vi "Stop Condition - Saturation 2 (SubVI) (1).vi"(6 "Enum":enum16{"Saturation", "Sat Step", "Sat Ramp"}(ring), 8 "error in (no error)":errorcluster, 9 "Test RunTime":dbl, 10 "Time":dbl, 11 "Cluster in":T1 {"M Event" items=["Stop", "Running", "PID", "Up Limit", "Down Limit", "Load Limit"]; "Test Type" items=["Please Select", "Triaxial Shear", "Triaxial UU", "Shearbox", "Permeability", "Consolidation (Stepped Loading)/Swelling", "Saturation (Incremental)", "User Defined", "UCT", "Isotropic Consolidation", "Swelling Pressure", "B-Check", "Saturation (Step Increment)", "Saturation (Ramp)"]; "Data"."Test Type" items=["Please Select", "Triaxial Shear", "Triaxial UU", "Shearbox", "Permeability", "Consolidation (Stepped Loading)/Swelling", "Saturation (Incremental)", "User Defined", "UCT", "Isotropic Consolidation", "Swelling Pressure", "B-Check", "Saturation (Step Increment)", "Saturation (Ramp)"]}) -> (0 "error out":errorcluster, 3 "Cluster out":T1 {"M Event" items=["Stop", "Running", "PID", "Up Limit", "Down Limit", "Load Limit"]; "Test Type" items=["Please Select", "Triaxial Shear", "Triaxial UU", "Shearbox", "Permeability", "Consolidation (Stepped Loading)/Swelling", "Saturation (Incremental)", "User Defined", "UCT", "Isotropic Consolidation", "Swelling Pressure", "B-Check", "Saturation (Step Increment)", "Saturation (Ramp)"]; "Data"."Test Type" items=["Please Select", "Triaxial Shear", "Triaxial UU", "Shearbox", "Permeability", "Consolidation (Stepped Loading)/Swelling", "Saturation (Incremental)", "User Defined", "UCT", "Isotropic Consolidation", "Swelling Pressure", "B-Check", "Saturation (Step Increment)", "Saturation (Ramp)"]}, 4 "Delay":string, 7 "Log?":bool)   [LabVIEW 2019]
uses:
  Controls/RunTest - Data Structure.ctl
  Controls/Test Panel - Data Structure.ctl
  Controls/Station - Test Type.ctl
  <vilib>/Utility/miscctls.llb/LVRowAndColumnTypeDef.ctl
  Controls/RunTest - Calculate Data.ctl
  <vilib>/httpClient/ClientHandle.ctl
  Controls/RunTest - Start Condition.ctl
  Controls/RunTest - Stop Condition.ctl
  Controls/UDP - Event.ctl
  Controls/eFGV States.ctl
  <vilib>/httpClient/LabVIEWHTTPClient.lvlib
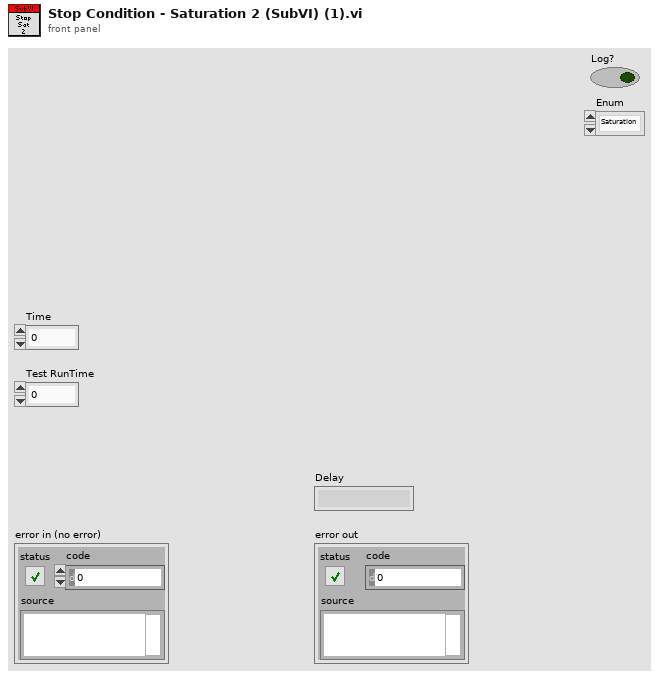
[diagram p1: front panel]
types:
  T1 = typedef "RunTest - Data Structure.ctl" = cluster{"Test Plan":string[], "PlanRow":i32, "Device Name":string[], "Timeout":i32, "Start?":bool, "Pause?":bool, "IP Address":string[], "LogRow":i32, "Logtype":u16, "Log Elapse":sgl, "Data":T2, "Stop log?":bool, "tdms":refnum<k34>, "Sensor Data":sgl[], "Start time":timestamp, "Prev Log Elapse":u32, "Plot":u16, "X-Axis":u16[], "Y-Axis":u16[], "XY":cluster{"X":dbl, "Y":dbl}[][], "End Stage?":bool, "1run":bool, "Condition":u16[], "Start Con":bool, "Log Con":bool, "Stop Con":bool, "Start Elapse":dbl, "Start Load":dbl, "Motor":i32, "StartRow":i32, "number log":i32, "Dir":bool, "Start time test":timestamp, "Auto":bool, "Check return?":bool, "Inv":cluster{"M":i32[], "Bool":bool[]}, "tdms temp":refnum<k34>, "Zero?":bool, "Plot Timer":dbl, "1st Run":bool, "TDMS Path":path, "MaxLoad":dbl, "Log Timer":sgl[], "Test Type":T3, "Log Sensor":string[], "Save?":bool, "1st Log":bool, "Y-Axis 2":u16[], "On Y-Axis 2":bool, "Decimal":u8[], "Init":cluster{"PWP TS":sgl, "Load TS":sgl, "Volume TS":sgl, "Disp TS":sgl, "CP":sgl, "Vol In":sgl, "Vol Out":sgl, "Load UCT":sgl, "Disp UCT":sgl, "PWP Sat":sgl, "CP Sat":sgl, "Volume IsoCons":sgl, "PWP IsoCons":sgl, "PWP TUU":sgl, "Load TUU":sgl, "Volume TUU":sgl, "Disp TUU":sgl, "Load Cons":sgl, "Disp Cons":sgl, "Volume Sat":sgl, "Vertical Load SB":sgl, "Vertical Disp SB":sgl, "H Disp SB":sgl, "H Load SB":sgl, "PWP BC":sgl, "CP BC":sgl, "PWP Sat Step":sgl, "CP Sat Step":sgl, "Volume Sat Step":sgl, "PWP Sat Ramp":sgl, "CP Sat Ramp":sgl, "Volume Sat Ramp":sgl}, "Calc":T5, "Device Index":i32[], "Channel Index":i32[], "http ref":T6, "fileid":string, "Step Cons":cluster{"V Stress":sgl, "H Settlement":sgl}, "RunTest":bool, "Graph Last":i32, "Init?":bool, "Datalog":bool[], "Start":T7, "Stop":T8, "Running?":bool, "StartTime":dbl, "Log Prev Time":dbl, "KeyName":string[], "Test RunTime":dbl, "Log Prev Axial":dbl, "M Event":T9[], "Last Log":bool, "popup":bool, "PreStart UU":bool, "PreStart Sat":bool, "PreStart BC":bool, "PreStart Sat Step":bool, "PreStart Sat Ramp":bool, "Prev Sat IP":string}
  T2 = typedef "Test Panel - Data Structure.ctl" = cluster{"Station":string, "Sample ID":string, "Job No":string, "Job Description":string, "Filename":string, "Test Type":T3, "Speciment No":string, "Depth":string, "Height":string, "Diameter/Length":string, "Weight":string, "Test Parameter":string, "Station[]":string[], "Edit Pos":T4, "Edit Pos Prev":T4, "Area":string, "Path":string, "sample_id":string}
  T3 = typedef "Station - Test Type.ctl" = u16
  T4 = typedef "LVRowAndColumnTypeDef.ctl" = cluster{"Row":i32, "Column":i32}
  T5 = typedef "RunTest - Calculate Data.ctl" = cluster{"TS":cluster{"Change PWP":sgl, "Change Vol":sgl, "Axial Load":sgl, "CiL":sgl, "Deviator":sgl, "Axial Strain":sgl, "MaxDeviator":sgl, "SS":sgl, "CAS":sgl}, "TUU":cluster{"Change PWP":sgl, "Axial Load":sgl, "CiL":sgl, "Deviator":sgl, "Axial Strain":sgl, "MaxDeviator":sgl}, "Sat":cluster{"B Value":sgl, "PWP Diss":sgl, "CPP":sgl, "CV":sgl}, "Per":cluster{"Change Vol In":sgl, "Change Vol Out":sgl, "Mean Vol":sgl, "Gradient Pressure":sgl, "Outlet Flow":sgl, "Inlet Flow":sgl, "I X1":sgl, "I X2":sgl, "I Y1":sgl, "I Y2":sgl, "O X1":sgl, "O X2":sgl, "O Y1":sgl, "O Y2":sgl}, "Step Cons":cluster{"V Stress":sgl, "H Settlement":sgl, "Total H Settle":sgl, "Prev Total H":sgl}, "UCT":cluster{"ALC":sgl, "H Change":sgl, "Deviator":sgl, "Axial Strain":sgl, "V Stress":sgl, "MaxDeviator":sgl}, "ISO Cons":cluster{"CPP":sgl, "PWP Diss":sgl, "CV":sgl, "VS":sgl}, "SB":cluster{"Speci LenC":sgl, "Shear Strain":sgl, "H LC":sgl, "Normal Stress":sgl, "Shear Stress":sgl, "MaxShear":sgl}, "BC":cluster{"B Value":sgl, "PWP Diss":sgl, "CPP":sgl, "CV":sgl}, "Sat Step":cluster{"B Value":sgl, "PWP Diss":sgl, "CPP":sgl, "CV":sgl}, "Sat Ramp":cluster{"B Value":sgl, "PWP Diss":sgl, "CPP":sgl, "CV":sgl}, "Prev Log":string[]}
  T6 = typedef "LabVIEWHTTPClient.lvlib/ClientHandle.ctl" = refnum<k1>
  T7 = typedef "RunTest - Start Condition.ctl" = cluster{"Cons":cluster{"VS":dbl, "Delay":bool, "No Delay":dbl}, "Sat":cluster{"CP":dbl, "BP":dbl, "StartBP":bool, "Target CP":bool, "Target BP":bool}, "Iso":cluster{"Select":dbl, "BP":dbl, "IC2":dbl, "IC3":dbl, "IC4":dbl, ". IC6":bool, "IC6":dbl, "IC6-2":dbl, "Time Cond":dbl, "Last PWP":dbl, "Target CP":bool, "Target BP":bool, "NewCP":dbl, "NewBP":dbl, "Noti CP":bool, "Noti BP":bool, "Noti PWP":bool, "PrevSatBP":dbl}, "TS":cluster{"SS":dbl, "Engage":bool, "ES":dbl, "LC":dbl, "PreStart":bool, "Trig SS":bool, "Drain":dbl, "Select":u16, "Max SS .":bool, "MaxSS":dbl}, "TUU":cluster{"SS":dbl, "Engage":bool, "ES":dbl, "LC":dbl, "PreStart":bool, "Trig SS":bool, "CP":dbl, "Delay Value":dbl, "Delay":bool, "CP PID":bool}, "UCT":cluster{"SS":dbl, "Engage":bool, "ES":dbl, "LC":dbl, "PreStart":bool, "Trig SS":bool}, "Enable?":bool, "SB":cluster{"SS":dbl, "Engage":bool, "ES":dbl, "LC":dbl, "PreStart":bool, "Trig SS":bool, "VS":dbl, "Delay Value":dbl, "Delay":bool, "VS PID":bool}, "Perm":cluster{"DP":dbl}, "BC":cluster{"CP":dbl, "Target CP":bool, "Target BP":bool, "CP Inc":dbl, "CP .Init":bool, "CP Init":dbl, "1st BC":bool}, "Sat (Step)":cluster{"Select":dbl, "CP":dbl, "BP":dbl, "EP":dbl, "StartCP":bool, "Target CP":bool, "Target BP":bool}, "Sat (Ramp)":cluster{"Select":dbl, "CP":dbl, "BP":dbl, "EP":dbl, "StartCP":bool, "Target CP":bool, "Target BP":bool, "Time Rate":u32}}
  T8 = typedef "RunTest - Stop Condition.ctl" = cluster{"Cons":cluster{"Select":i32, "Disp":dbl, "Time":dbl, "Time2":dbl, "Disp 2":dbl, "Time Cond":dbl, "Last Disp":dbl, "Swell":bool, "T50,90,100":cluster{"t50_x_min":dbl, "t50_y_value":dbl, "t90_x_min":dbl, "t90_y_value":dbl, "t100_x_min":dbl, "t100_y_value":dbl, "target_column":string, "test_type":string, "error":string}}, "Sat":cluster{"Select":i32, "PP":dbl, "Time":dbl, "VC":dbl, "Time2":dbl, "Time Cond":dbl, "Last PP":dbl, ".B":bool, "B":dbl, "Last Vc":dbl, "Time Cond 2":dbl, "Time3":dbl, "Time Cond 3":dbl, "B Achieve":bool, "PP Achieve":bool, "VC Achieve":bool, "Max Achieve":bool, "CP Check":dbl, "Skip Next":bool, "B Achieve Stage":u32, ".CP Check":bool}, "Iso":cluster{"PP":dbl, "Time":dbl, "VC":dbl, "Time2":dbl, "Time Cond":dbl, "Last Vc":dbl, ".PP":bool, "Time Cond 2":dbl, "Select":i32, "BS":cluster{"t50_x_min":dbl, "t50_y_value":dbl, "t90_x_min":dbl, "t90_y_value":dbl, "t100_x_min":dbl, "t100_y_value":dbl, "target_column":string, "test_type":string, "error":string}, "Final VC":dbl, "ASTM":cluster{"t50_x_min":dbl, "t50_y_value":dbl, "t90_x_min":dbl, "t90_y_value":dbl, "t100_x_min":dbl, "t100_y_value":dbl, "target_column":string, "test_type":string, "error":string}, "ASTM Log":cluster{"t50_x_min":dbl, "t50_y_value":dbl, "t90_x_min":dbl, "t90_y_value":dbl, "t100_x_min":dbl, "t100_y_value":dbl, "target_column":string, "test_type":string, "error":string}, "PP Achieve":bool, "VC Achieve":bool}, "TS":cluster{"Axial":dbl, ".MaxDev":bool, "MaxDev Value":dbl, "Return":bool, "Reset":bool, "Prev Time":dbl, "PostStop Run":bool, "CP Stop":bool, "BP Stop":bool, "PostStop Trig":bool, "Reset Value":dbl, "BPTrig":bool, "CPTrig":bool, "VLCTrig":bool, "CAxial":dbl, "Select":i32}, "TUU":cluster{"Axial":dbl, ".MaxDev":bool, "MaxDev Value":dbl, "Return":bool, "Reset":bool, "Prev Time":dbl, "PostStop Run":bool, "CP Stop":bool, "BP Stop":bool, "PostStop Trig":bool, "Reset Value":dbl, "BPTrig":bool, "CPTrig":bool, "VLCTrig":bool}, "UCT":cluster{"Axial":dbl, ".MaxDev":bool, "MaxDev Value":dbl, "Return":bool, "Reset":bool, "Prev Time":dbl, "PostStop Run":bool, "CP Stop":bool, "BP Stop":bool, "PostStop Trig":bool}, "Enable?":bool, "SB":cluster{"Shear":dbl, ".MaxShear":bool, "MaxShear Value":dbl, "Return":bool, "Reset":bool, "Prev Time":dbl, "PostStop Run":bool, "CP Stop":bool, "BP Stop":bool, "PostStop Trig":bool, "Reset Value":dbl, "BPTrig":bool, "CPTrig":bool, "VLCTrig":bool}, "Perm":cluster{"Max Time":bool, "Reset":bool, "PostStop Run":bool, "Ratio":bool, "Reset Value":dbl, "Time":dbl, "RatioTime":dbl, "RatioMore":dbl, "RatioLess":dbl, "Time Cond":dbl, "Time Cond 2":dbl, "Prev IF":dbl, "Prev OF":dbl, "PostStop Trig":bool, "BP Trig":bool, "DP Stop":bool, "BP Stop":bool, "CP Stop":bool, "CP Trig":bool}, "SP":cluster{".Max Time":bool, ".Time":bool, "Time":dbl, "MaxTime":dbl, "Time Cond":dbl, "Max Time Cond":dbl, "Stress":dbl}, "BC":cluster{"Select":i32, "PP":dbl, "Time":dbl, "Time Cond":dbl, "Last PP":dbl, ".B":bool, "B":dbl, "Time 2":dbl, "Time Cond 2":dbl, "B Achieve":bool, "PP Achieve":bool, "Max Achieve":bool, "CP Check":dbl, "Skip Next":bool, "B Achieve Stage":u32, ".CP Check":bool}, "Sat (Step)":cluster{"Select":i32, "PP":dbl, "Time":dbl, "VC":dbl, "Time2":dbl, "Time Cond":dbl, "Last PP":dbl, ".B":bool, "B":dbl, "Last Vc":dbl, "Time Cond 2":dbl, "Time3":dbl, "Time Cond 3":dbl, "B Achieve":bool, "PP Achieve":bool, "VC Achieve":bool, "Max Achieve":bool, "CP Check":dbl, "Skip Next":bool, "B Achieve Stage":u32}, "Sat (Ramp)":cluster{"Select":i32, "PP":dbl, "Time":dbl, "VC":dbl, "Time2":dbl, "Time Cond":dbl, "Last PP":dbl, ".B":bool, "B":dbl, "Last Vc":dbl, "Time Cond 2":dbl, "Time3":dbl, "Time Cond 3":dbl, "B Achieve":bool, "PP Achieve":bool, "VC Achieve":bool, "Max Achieve":bool, "CP Check":dbl, "Skip Next":bool, "B Achieve Stage":u32}}
  T9 = typedef "UDP - Event.ctl" = u16
  T10 = typedef "eFGV States.ctl" = enum16{"Init", "Read", "Write", "Exit"}
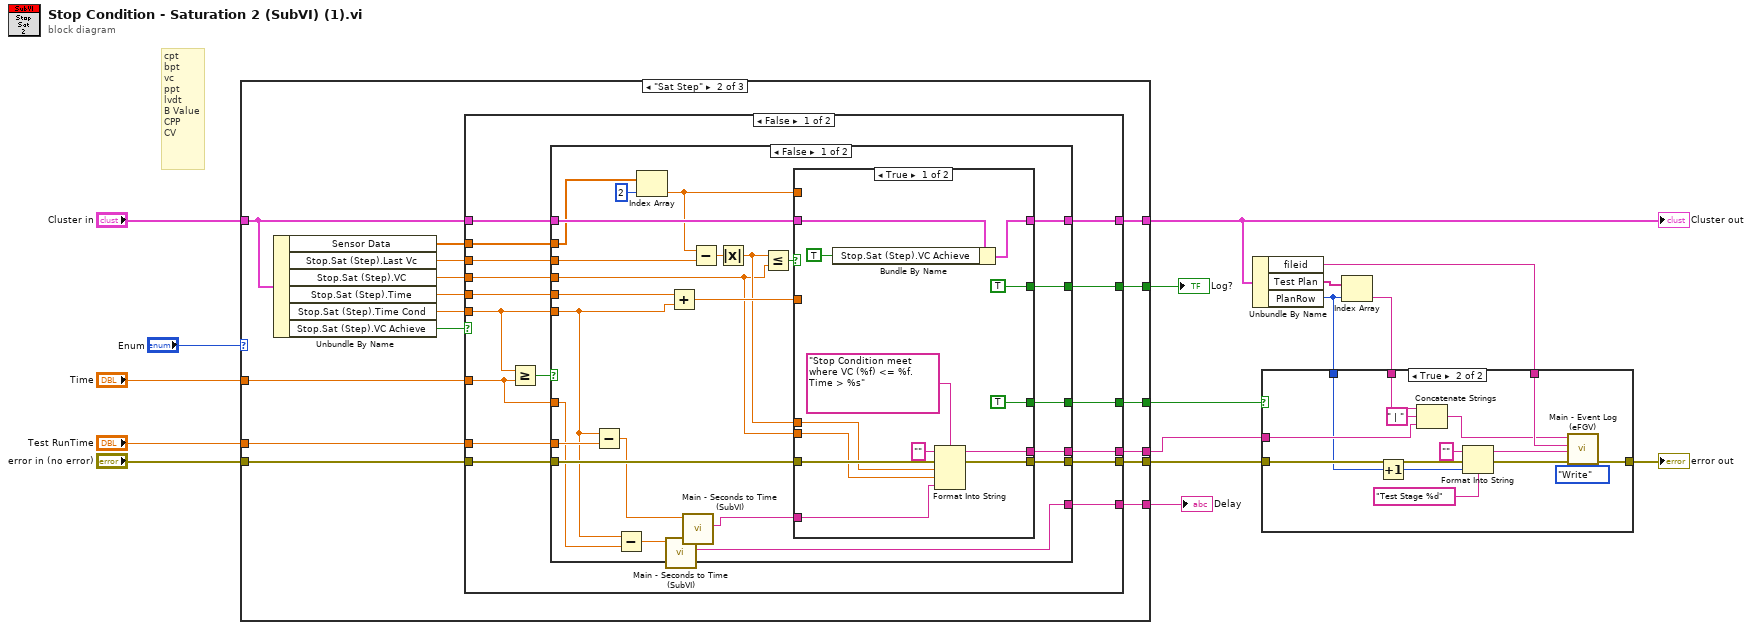
[diagram p0: block diagram]
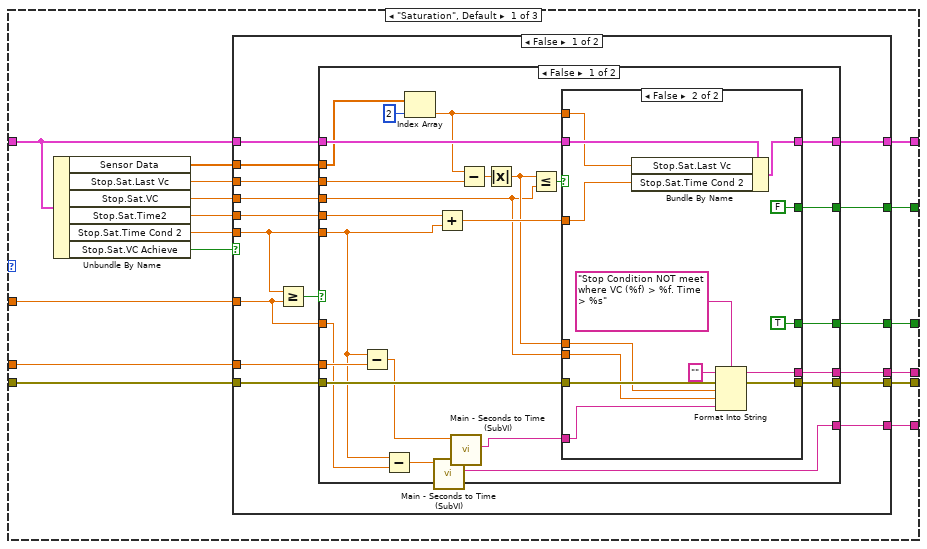
[diagram p2: hidden frame]
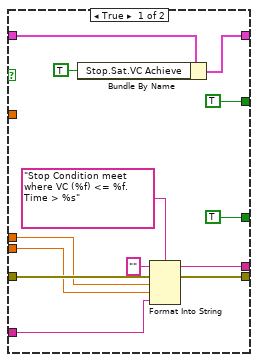
[diagram p3: hidden frame]
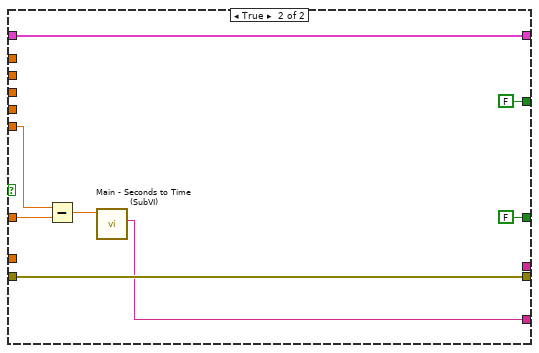
[diagram p4: hidden frame]
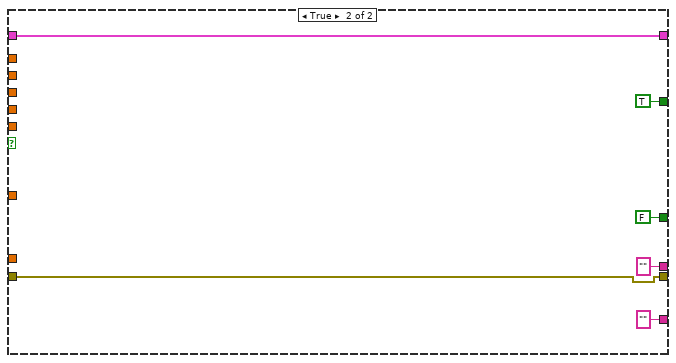
[diagram p5: hidden frame]
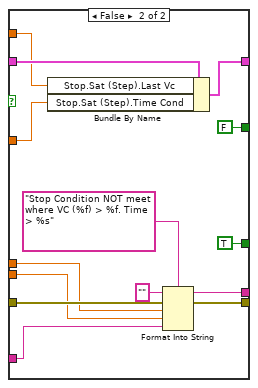
[diagram p6: hidden frame]
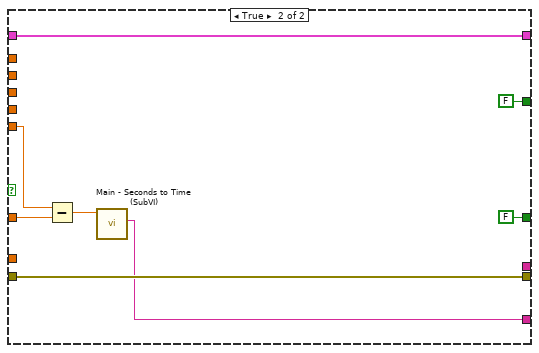
[diagram p7: hidden frame]
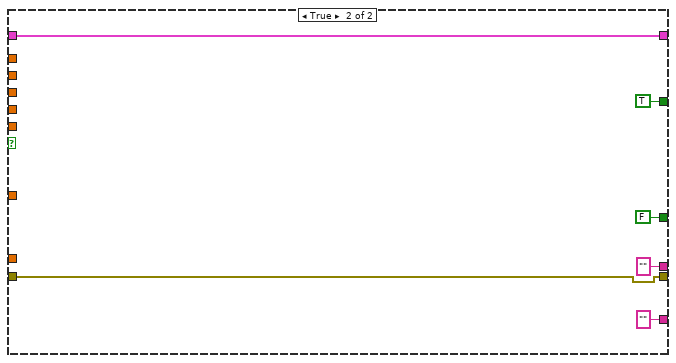
[diagram p8: hidden frame]
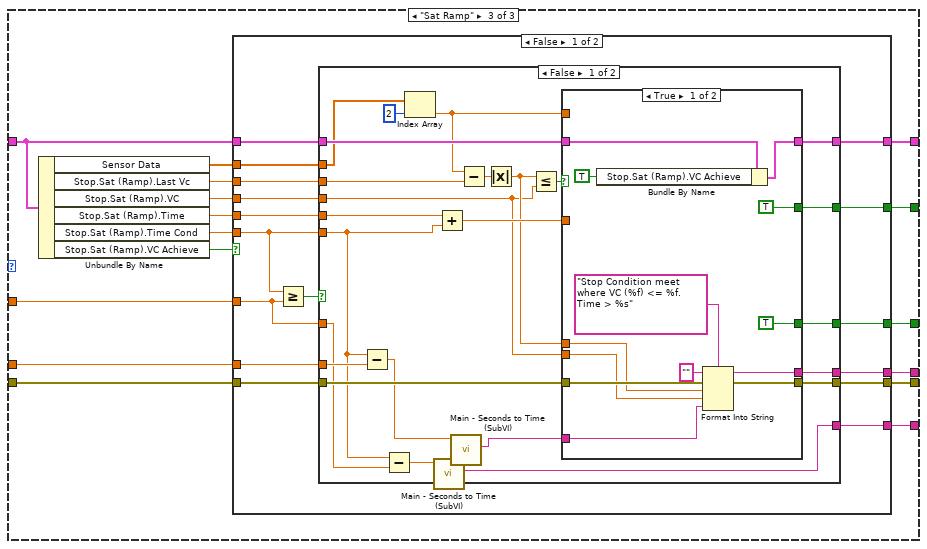
[diagram p9: hidden frame]
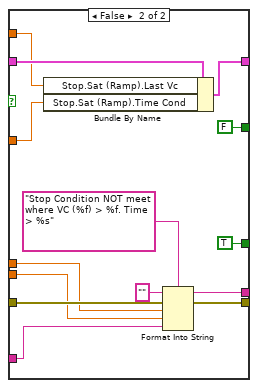
[diagram p10: hidden frame]
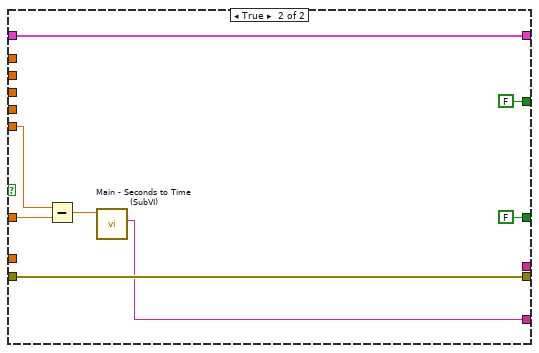
[diagram p11: hidden frame]
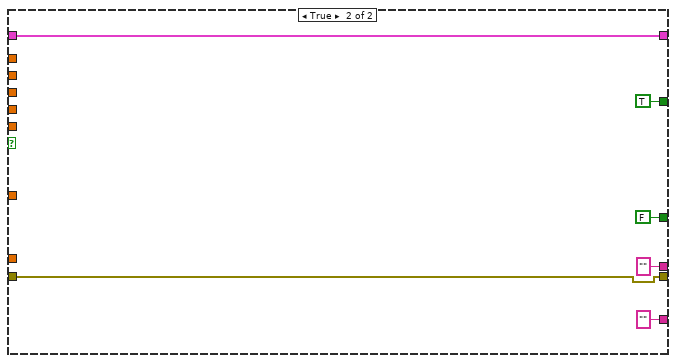
[diagram p12: hidden frame]
diagram:
  # "cpt\nbpt\nvc\nppt\nlvdt\nB Value\nCPP\nCV"
  n1 = case shown="\"Sat Step\"" "Enum" {
    tunnel: [w32 w129 w226] -> w16
    tunnel: "Cluster in" -> [w26 w123 w220]
    tunnel: "Test RunTime" -> [w25 w122 w219]
    tunnel: "Time" -> [w24 w121 w218]
    tunnel: "error in (no error)" -> [w23 w120 w217]
    tunnel: [w22 w119 w216] -> w11
    tunnel: [w20 w117 w214] -> w6
    tunnel: [w19 w116 w213] -> w5
    tunnel: [w18 w115 w212] -> w4
    tunnel: [w17 w114 w211] -> w3
    frame "Saturation", Default {
      n2 = Unbundle By Name(w26) -> ("Sensor Data"=w27:sgl[], "Stop.Sat.Last Vc"=w28:dbl, "Stop.Sat.VC"=w29:dbl, "Stop.Sat.Time2"=w30:dbl, "Stop.Sat.Time Cond 2"=w31:dbl, "Stop.Sat.VC Achieve"=w21:bool)
      n3 = case shown="False" w21 {
        tunnel: [w48 "" ("Time string")] -> w32
        tunnel: w31 -> [w47 _]
        tunnel: w30 -> [w46 _]
        tunnel: w29 -> [w45 _]
        tunnel: w28 -> [w44 _]
        tunnel: w27 -> [w43 _]
        tunnel: w26 -> [w42 w113]
        tunnel: w25 -> [w41 _]
        tunnel: w24 -> [w40 _]
        tunnel: [w39 FALSE] -> w19
        tunnel: [w38 ""] -> w18
        tunnel: w23 -> [w37 w109]
        tunnel: [w35 w113] -> w17
        tunnel: [w34 w109] -> w20
        tunnel: [w33 TRUE] -> w22
        frame False {
          n4 = Greater Or Equal?(x=w47, y=w40) -> (x >= y?=w36:bool)
          n5 = case shown="False" w36 {
            tunnel: [w61 w107] -> w34
            tunnel: w37 -> [w62 w107]
            tunnel: [w72 w106] -> w35
            tunnel: w42 -> [w71 w106]
            tunnel: w44 -> [w68 _]
            tunnel: w45 -> [w57 _]
            tunnel: w46 -> [w70 _]
            tunnel: w47 -> [w52 w103]
            tunnel: w43 -> [w65 _]
            tunnel: [w60 _] -> w38
            tunnel: [w59 FALSE] -> w39
            tunnel: w40 -> [w51 w102]
            tunnel: w41 -> [w56 _]
            tunnel: [w50 w101] -> w48
            tunnel: [w49 FALSE] -> w33
            frame False {
              n6 = Subtract(x=w52, y=w56) -> (x-y=w55:dbl)
              n7 = Subtract(x=w52, y=w51) -> (x-y=w53:dbl)
              n8 = Index Array(array=w65, index=2) -> (element=w64:sgl)
              n9 = call "Main - Seconds to Time (SubVI).vi"("Seconds"=w53) -> ("Time string"=w50:string)  [unwired: 9 in, 1 out]
              n10 = Add(x=w70, y=w52) -> (x+y=w69:dbl)
              n11 = call "Main - Seconds to Time (SubVI).vi"("Seconds"=w55) -> ("Time string"=w54:string)  [unwired: 9 in, 1 out]
              n12 = Subtract(x=w64, y=w68) -> (x-y=w67:dbl)
              n13 = Absolute Value(x=w67) -> (abs(x)=w58:dbl)
              n14 = Less Or Equal?(x=w58, y=w57) -> (x <= y?=w66:bool)
              n15 = case shown="False" w66 {
                tunnel: [w74 w99] -> w72
                tunnel: w71 -> [w73 w98]
                tunnel: w69 -> [_ w97]
                tunnel: w64 -> [_ w96]
                tunnel: w62 -> [w84 w92]
                tunnel: [w83 w93] -> w61
                tunnel: [w82 w88] -> w60
                tunnel: [TRUE TRUE] -> w59
                tunnel: w54 -> [w80 w89]
                tunnel: w58 -> [w79 w91]
                tunnel: w57 -> [w78 w90]
                tunnel: [TRUE FALSE] -> w49
                frame True {
                  n16 = Bundle By Name(cluster=w73, "Stop.Sat.VC Achieve"=TRUE) -> (w74:T1)
                  n17 = Format Into String(format string="Stop Condition meet where VC (%f) <= %f. Time > %s", initial string="", error in=w84, w79, w78, w80) -> (resulting string=w82:string, error out=w83:errorcluster)
                }
                frame False {
                  n18 = Bundle By Name(cluster=w98, "Stop.Sat.Last Vc"=w96, "Stop.Sat.Time Cond 2"=w97) -> (w99:T1)
                  n19 = Format Into String(format string="Stop Condition NOT meet where VC (%f) > %f. Time > %s", initial string="", error in=w92, w91, w90, w89) -> (resulting string=w88:string, error out=w93:errorcluster)
                }
              }
            }
            frame True {
              n20 = Subtract(x=w103, y=w102) -> (x-y=w104:dbl)
              n21 = call "Main - Seconds to Time (SubVI).vi"("Seconds"=w104) -> ("Time string"=w101:string)  [unwired: 9 in, 1 out]
            }
          }
        }
        frame True {
        }
      }
    }
    frame "Sat Step" {
      n22 = Unbundle By Name(w123) -> ("Sensor Data"=w124:sgl[], "Stop.Sat (Step).Last Vc"=w125:dbl, "Stop.Sat (Step).VC"=w126:dbl, "Stop.Sat (Step).Time"=w127:dbl, "Stop.Sat (Step).Time Cond"=w128:dbl, "Stop.Sat (Step).VC Achieve"=w118:bool)
      n23 = case shown="False" w118 {
        tunnel: [w145 "" ("Time string")] -> w129
        tunnel: w128 -> [w144 _]
        tunnel: w127 -> [w143 _]
        tunnel: w126 -> [w142 _]
        tunnel: w125 -> [w141 _]
        tunnel: w124 -> [w140 _]
        tunnel: w123 -> [w139 w210]
        tunnel: w122 -> [w138 _]
        tunnel: w121 -> [w137 _]
        tunnel: [w136 FALSE] -> w116
        tunnel: [w135 ""] -> w115
        tunnel: w120 -> [w134 w206]
        tunnel: [w132 w210] -> w114
        tunnel: [w131 w206] -> w117
        tunnel: [w130 TRUE] -> w119
        frame False {
          n24 = Greater Or Equal?(x=w144, y=w137) -> (x >= y?=w133:bool)
          n25 = case shown="False" w133 {
            tunnel: [w158 w204] -> w131
            tunnel: w134 -> [w159 w204]
            tunnel: [w169 w203] -> w132
            tunnel: w139 -> [w168 w203]
            tunnel: w141 -> [w165 _]
            tunnel: w142 -> [w154 _]
            tunnel: w143 -> [w167 _]
            tunnel: w144 -> [w149 w200]
            tunnel: w140 -> [w162 _]
            tunnel: [w157 _] -> w135
            tunnel: [w156 FALSE] -> w136
            tunnel: w137 -> [w148 w199]
            tunnel: w138 -> [w153 _]
            tunnel: [w147 w198] -> w145
            tunnel: [w146 FALSE] -> w130
            frame False {
              n26 = Subtract(x=w149, y=w153) -> (x-y=w152:dbl)
              n27 = Subtract(x=w149, y=w148) -> (x-y=w150:dbl)
              n28 = Index Array(array=w162, index=2) -> (element=w161:sgl)
              n29 = call "Main - Seconds to Time (SubVI).vi"("Seconds"=w150) -> ("Time string"=w147:string)  [unwired: 9 in, 1 out]
              n30 = Add(x=w167, y=w149) -> (x+y=w166:dbl)
              n31 = call "Main - Seconds to Time (SubVI).vi"("Seconds"=w152) -> ("Time string"=w151:string)  [unwired: 9 in, 1 out]
              n32 = Subtract(x=w161, y=w165) -> (x-y=w164:dbl)
              n33 = Absolute Value(x=w164) -> (abs(x)=w155:dbl)
              n34 = Less Or Equal?(x=w155, y=w154) -> (x <= y?=w163:bool)
              n35 = case shown="True" w163 {
                tunnel: [w171 w196] -> w169
                tunnel: w168 -> [w170 w195]
                tunnel: w166 -> [_ w194]
                tunnel: w161 -> [_ w193]
                tunnel: w159 -> [w181 w189]
                tunnel: [w180 w190] -> w158
                tunnel: [w179 w185] -> w157
                tunnel: [TRUE TRUE] -> w156
                tunnel: w151 -> [w177 w186]
                tunnel: w155 -> [w176 w188]
                tunnel: w154 -> [w175 w187]
                tunnel: [TRUE FALSE] -> w146
                frame True {
                  n36 = Bundle By Name(cluster=w170, "Stop.Sat (Step).VC Achieve"=TRUE ("Stop.Sat.VC Achieve")) -> (w171:T1)
                  n37 = Format Into String(format string="Stop Condition meet where VC (%f) <= %f. Time > %s", initial string="", error in=w181, w176, w175, w177) -> (resulting string=w179:string, error out=w180:errorcluster)
                }
                frame False {
                  n38 = Bundle By Name(cluster=w195, "Stop.Sat (Step).Last Vc"=w193, "Stop.Sat (Step).Time Cond"=w194) -> (w196:T1)
                  n39 = Format Into String(format string="Stop Condition NOT meet where VC (%f) > %f. Time > %s", initial string="", error in=w189, w188, w187, w186) -> (resulting string=w185:string, error out=w190:errorcluster)
                }
              }
            }
            frame True {
              n40 = Subtract(x=w200, y=w199) -> (x-y=w201:dbl)
              n41 = call "Main - Seconds to Time (SubVI).vi"("Seconds"=w201) -> ("Time string"=w198:string)  [unwired: 9 in, 1 out]
            }
          }
        }
        frame True {
        }
      }
    }
    frame "Sat Ramp" {
      n42 = Unbundle By Name(w220) -> ("Sensor Data"=w221:sgl[], "Stop.Sat (Ramp).Last Vc"=w222:dbl, "Stop.Sat (Ramp).VC"=w223:dbl, "Stop.Sat (Ramp).Time"=w224:dbl, "Stop.Sat (Ramp).Time Cond"=w225:dbl, "Stop.Sat (Ramp).VC Achieve"=w215:bool)
      n43 = case shown="False" w215 {
        tunnel: [w242 "" ("Time string")] -> w226
        tunnel: w225 -> [w241 _]
        tunnel: w224 -> [w240 _]
        tunnel: w223 -> [w239 _]
        tunnel: w222 -> [w238 _]
        tunnel: w221 -> [w237 _]
        tunnel: w220 -> [w236 w307]
        tunnel: w219 -> [w235 _]
        tunnel: w218 -> [w234 _]
        tunnel: [w233 FALSE] -> w213
        tunnel: [w232 ""] -> w212
        tunnel: w217 -> [w231 w303]
        tunnel: [w229 w307] -> w211
        tunnel: [w228 w303] -> w214
        tunnel: [w227 TRUE] -> w216
        frame False {
          n44 = Greater Or Equal?(x=w241, y=w234) -> (x >= y?=w230:bool)
          n45 = case shown="False" w230 {
            tunnel: [w255 w301] -> w228
            tunnel: w231 -> [w256 w301]
            tunnel: [w266 w300] -> w229
            tunnel: w236 -> [w265 w300]
            tunnel: w238 -> [w262 _]
            tunnel: w239 -> [w251 _]
            tunnel: w240 -> [w264 _]
            tunnel: w241 -> [w246 w297]
            tunnel: w237 -> [w259 _]
            tunnel: [w254 _] -> w232
            tunnel: [w253 FALSE] -> w233
            tunnel: w234 -> [w245 w296]
            tunnel: w235 -> [w250 _]
            tunnel: [w244 w295] -> w242
            tunnel: [w243 FALSE] -> w227
            frame False {
              n46 = Subtract(x=w246, y=w250) -> (x-y=w249:dbl)
              n47 = Subtract(x=w246, y=w245) -> (x-y=w247:dbl)
              n48 = Index Array(array=w259, index=2) -> (element=w258:sgl)
              n49 = call "Main - Seconds to Time (SubVI).vi"("Seconds"=w247) -> ("Time string"=w244:string)  [unwired: 9 in, 1 out]
              n50 = Add(x=w264, y=w246) -> (x+y=w263:dbl)
              n51 = call "Main - Seconds to Time (SubVI).vi"("Seconds"=w249) -> ("Time string"=w248:string)  [unwired: 9 in, 1 out]
              n52 = Subtract(x=w258, y=w262) -> (x-y=w261:dbl)
              n53 = Absolute Value(x=w261) -> (abs(x)=w252:dbl)
              n54 = Less Or Equal?(x=w252, y=w251) -> (x <= y?=w260:bool)
              n55 = case shown="True" w260 {
                tunnel: [w268 w293] -> w266
                tunnel: w265 -> [w267 w292]
                tunnel: w263 -> [_ w291]
                tunnel: w258 -> [_ w290]
                tunnel: w256 -> [w278 w286]
                tunnel: [w277 w287] -> w255
                tunnel: [w276 w282] -> w254
                tunnel: [TRUE TRUE] -> w253
                tunnel: w248 -> [w274 w283]
                tunnel: w252 -> [w273 w285]
                tunnel: w251 -> [w272 w284]
                tunnel: [TRUE FALSE] -> w243
                frame True {
                  n56 = Bundle By Name(cluster=w267, "Stop.Sat (Ramp).VC Achieve"=TRUE ("Stop.Sat.VC Achieve")) -> (w268:T1)
                  n57 = Format Into String(format string="Stop Condition meet where VC (%f) <= %f. Time > %s", initial string="", error in=w278, w273, w272, w274) -> (resulting string=w276:string, error out=w277:errorcluster)
                }
                frame False {
                  n58 = Bundle By Name(cluster=w292, "Stop.Sat (Ramp).Last Vc"=w290, "Stop.Sat (Ramp).Time Cond"=w291) -> (w293:T1)
                  n59 = Format Into String(format string="Stop Condition NOT meet where VC (%f) > %f. Time > %s", initial string="", error in=w286, w285, w284, w283) -> (resulting string=w282:string, error out=w287:errorcluster)
                }
              }
            }
            frame True {
              n60 = Subtract(x=w297, y=w296) -> (x-y=w298:dbl)
              n61 = call "Main - Seconds to Time (SubVI).vi"("Seconds"=w298) -> ("Time string"=w295:string)  [unwired: 9 in, 1 out]
            }
          }
        }
        frame True {
        }
      }
    }
  }
  "Delay" <- w16
  "Cluster out" <- w3
  "Log?" <- w11
  n62 = Unbundle By Name(w3) -> ("fileid"=w8:string, "Test Plan"=w9:string[], "PlanRow"=w7:i32)
  n63 = Index Array(array=w9, index=w7) -> (element=w10:string)
  n64 = case shown="True" w5 {
    tunnel: w6 -> [w308 w312]
    tunnel: [w308 w321] -> w2
    tunnel: w8 -> [_ w320]
    tunnel: w4 -> [_ w316]
    tunnel: w10 -> [_ w319]
    tunnel: w7 -> [_ w310]
    frame False {
    }
    frame True {
      n65 = Increment(x=w310) -> (x+1=w314:i32)
      n66 = Concatenate Strings(w319, " | " ("string"), w316) -> (w317:string)
      n67 = Format Into String(format string="Test Stage %d", initial string="", error in=w312, w314) -> (resulting string=w311:string, error out=w313:errorcluster)
      n68 = call "Main - Event Log (eFGV).vi"("Action"=eFGV_States."Write", "error in"=w313, "Stage"=w311, "Fileid"=w320, "Data In"=w317) -> ("error out"=w321:errorcluster)  [unwired: 3 in, 3 out]
    }
  }
  "error out" <- w2
